vi "voltage.vi"() -> ()   [LabVIEW 2019]
panel:
  in  "rate":dbl=1000.0
  in  "stop (F)":bool
  out "data":dynamicdata(graph)
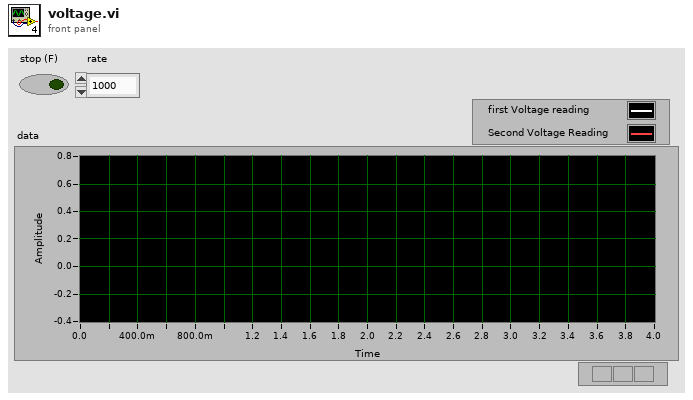
[diagram p1: front panel]
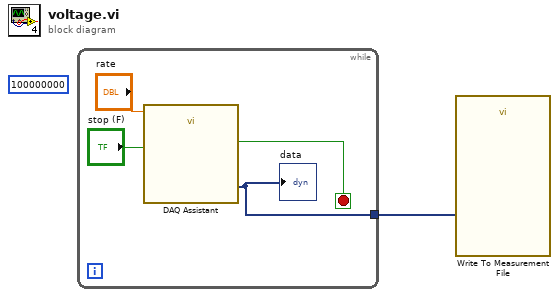
[diagram p0: block diagram]
diagram:
  (unwired) 100000000 ("number of samples")
  n1 = while {
    tunnel: [w2] -> w1
    stop <- w4 stop-if-true
    n2 = call "DAQ Assistant"("rate"="rate", "stop (F)"="stop (F)") -> ("data"=w2:dynamicdata, "stopped"=w4:bool)  [unwired: 14 in, 2 out]
    "data" <- w2
  }
  n3 = call "Write To Measurement File"("Signals"=w1) -> ()  [unwired: 16 in, 3 out]
